vi "Extract Segment.vi"(6 "Containing Type":T2, 8 "error in (no error)":errorcluster, 9 "In Type":bool, 10 "String":string, 11 "ProtoParser in":refnum<class "ProtoParser.lvclass">) -> (0 "error out":errorcluster, 1 "Segment":T1, 2 "Remaining":string, 3 "ProtoParser out":refnum<class "ProtoParser.lvclass">)   [LabVIEW 2020, in "LV-Protoc.lvlib" / "ProtoParser.lvclass"]
uses:
  ProtoParser.lvclass
  Segment Type.ctl
  Raw Segment.ctl
  ProtoParser.lvclass/ProtoParser.ctl
  LV-Protoc.lvlib
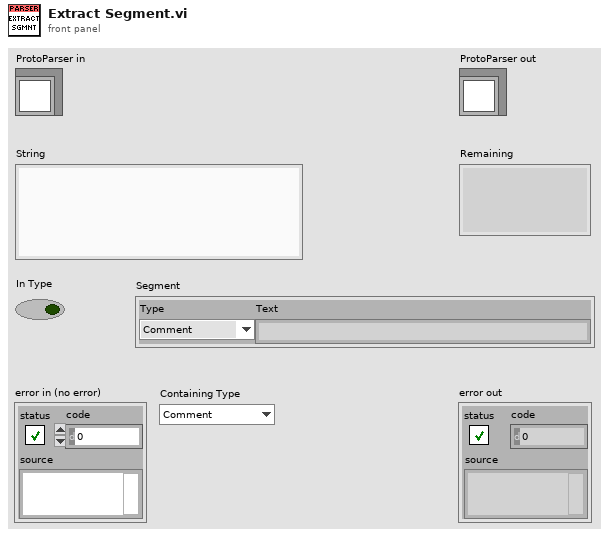
[diagram p1: front panel]
types:
  T1 = typedef "LV-Protoc.lvlib/Raw Segment.ctl" = cluster{"Type":T2, "Text":string}
  T2 = typedef "LV-Protoc.lvlib/Segment Type.ctl" = enum16{"Comment", "Message Open", "Enum Open", "Message Close", "Enum Close", "Field", "Syntax", "Import", "Enum Value", "Package", "Reserved"}
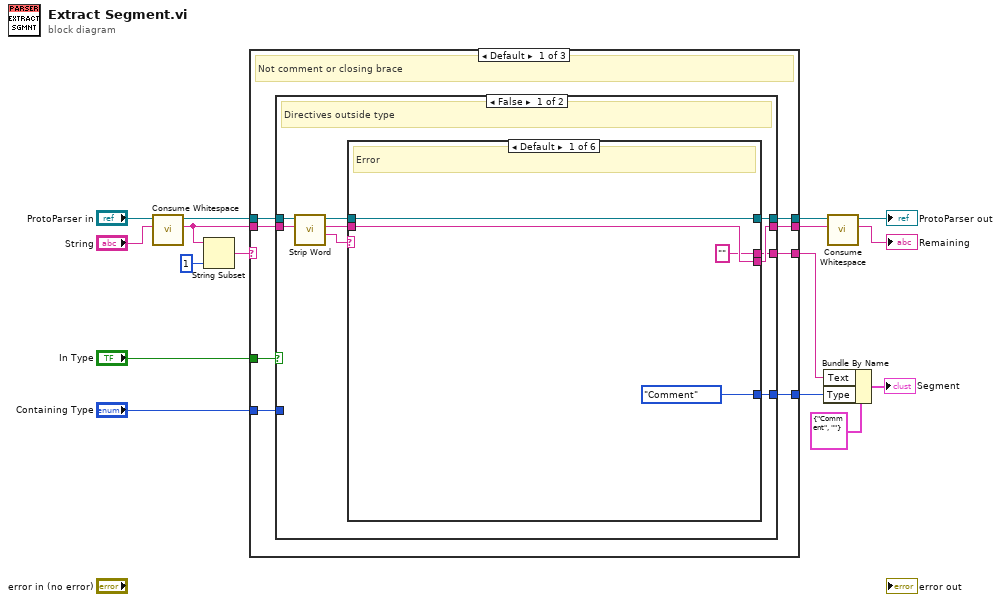
[diagram p0: block diagram]
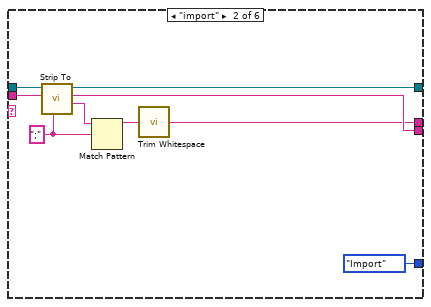
[diagram p2: hidden frame]
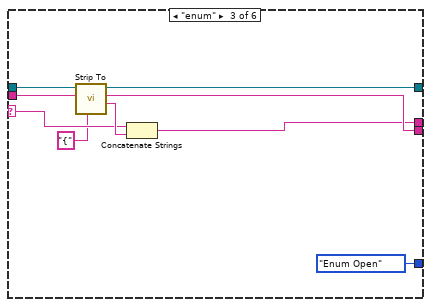
[diagram p3: hidden frame]
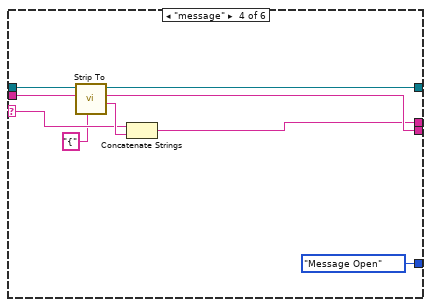
[diagram p4: hidden frame]
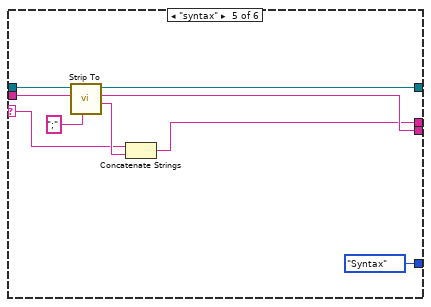
[diagram p5: hidden frame]
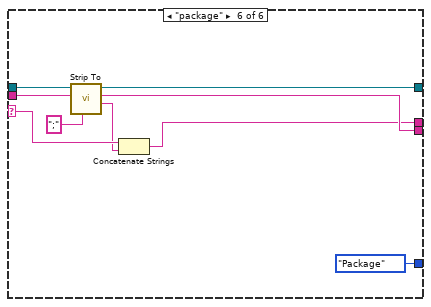
[diagram p6: hidden frame]
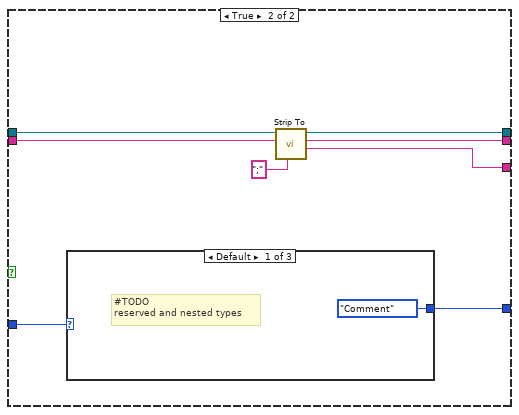
[diagram p7: hidden frame]
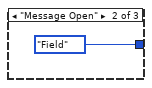
[diagram p8: hidden frame]
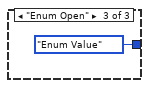
[diagram p9: hidden frame]
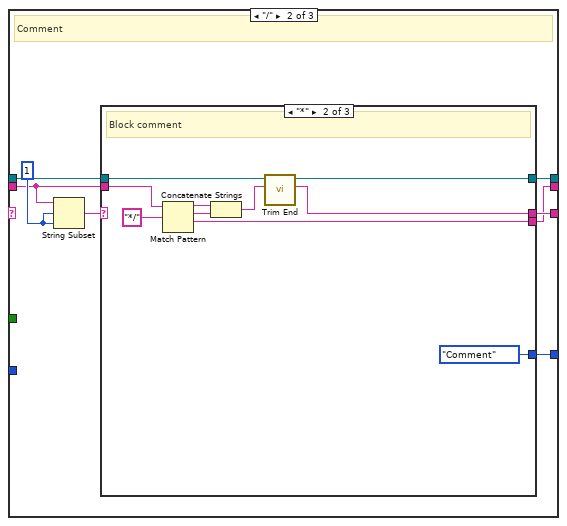
[diagram p10: hidden frame]
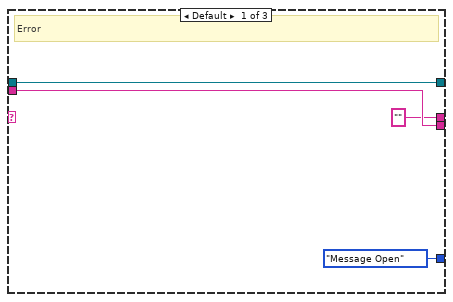
[diagram p11: hidden frame]
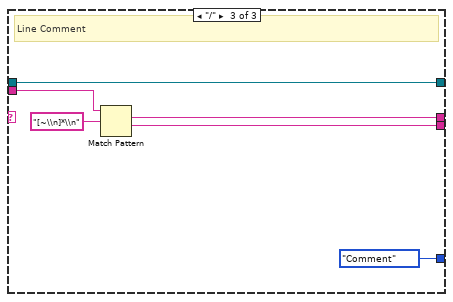
[diagram p12: hidden frame]
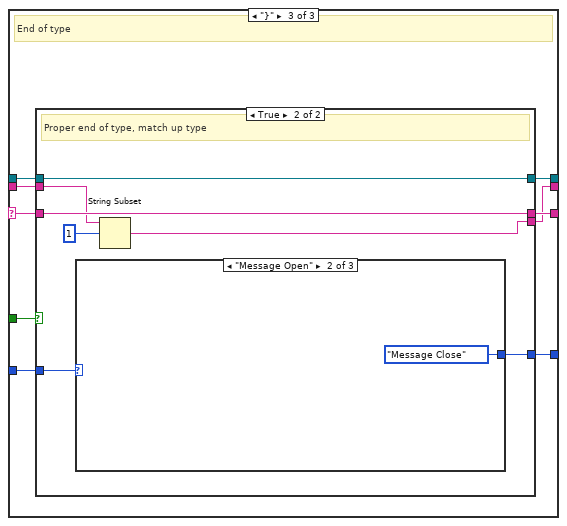
[diagram p13: hidden frame]
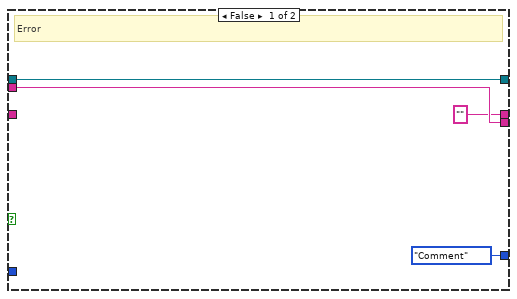
[diagram p14: hidden frame]
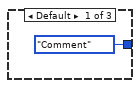
[diagram p15: hidden frame]
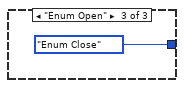
[diagram p16: hidden frame]
diagram:
  n1 = call "Consume Whitespace.vi"("String"="String", "ProtoParser in"="ProtoParser in") -> ("Remaining"=w11:string, "ProtoParser out"=w10:refnum<class "ProtoParser.lvclass">)  [unwired: 7 in, 1 out]
  n2 = String Subset(string=w11, length (rest)=1 ("length (rest)")) -> (substring=w13:string)  [unwired: 1 in]
  n3 = case shown="Default" w13 {
    selector: w13 -> [_ _ w125]
    tunnel: "In Type" -> [w24 _ w128]
    tunnel: w11 -> [w22 w99 w129]
    tunnel: [w18 w98 w124] -> w5
    tunnel: [w17 w97 w126] -> w6
    tunnel: [w19 w96 w122] -> w2
    tunnel: w10 -> [w23 w95 w130]
    tunnel: [w20 w94 w123] -> w4
    tunnel: "Containing Type" -> [w21 _ w127]
    frame Default {
      # "Not comment or closing brace"
      n4 = case shown="False" w24 {
        tunnel: w23 -> [w33 w86]
        tunnel: w22 -> [w32 w85]
        tunnel: w21 -> [_ w84]
        tunnel: [w28 w90] -> w20
        tunnel: [w27 w89] -> w19
        tunnel: [w26 w87] -> w18
        tunnel: [w25 w83] -> w17
        frame False {
          # "Directives outside type"
          n5 = call "Strip Word.vi"("String"=w32, "ProtoParser in"=w33) -> ("Word"=w29:string, "Remaining"=w30:string, "ProtoParser out"=w31:refnum<class "ProtoParser.lvclass">)  [unwired: 6 in, 1 out]
          n6 = case shown="Default" w29 {
            selector: w29 -> [_ _ w50 w59 w66 w76]
            tunnel: w31 -> [w37 w46 w55 w64 w73 w82]
            tunnel: w30 -> [w36 w45 w53 w62 w72 w81]
            tunnel: [w37 w43 w54 w63 w70 w79] -> w28
            tunnel: [w36 w44 w52 w61 w71 w80] -> w27
            tunnel: ["" w39 w49 w58 w65 w74] -> w26
            tunnel: [Segment_Type."Comment" ("Type") Segment_Type."Import" ("Type") Segment_Type."Enum Open" ("Type") Segment_Type."Message Open" ("Type") Segment_Type."Syntax" ("Type") Segment_Type."Package" ("Type")] -> w25
            frame Default {
              # "Error"
            }
            frame "import" {
              w41 = ";" ("End")
              n7 = call "Strip To.vi"("End"=w41, "String"=w45, "ProtoParser in"=w46) -> ("Portion"=w42:string, "Remaining"=w44:string, "ProtoParser out"=w43:refnum<class "ProtoParser.lvclass">)  [unwired: 5 in, 1 out]
              n8 = Match Pattern(string=w42, regular expression=w41) -> (before substring=w40:string)  [unwired: 1 in, 3 out]
              n9 = call <vilib>:"Trim Whitespace.vi"("string"=w40) -> ("trimmed string"=w39:string)  [unwired: 1 in]
            }
            frame "enum" {
              n10 = call "Strip To.vi"("End"="{", "String"=w53, "ProtoParser in"=w55) -> ("Portion"=w51:string, "Remaining"=w52:string, "ProtoParser out"=w54:refnum<class "ProtoParser.lvclass">)  [unwired: 5 in, 1 out]
              n11 = Concatenate Strings(w50, w51) -> (w49:string)
            }
            frame "message" {
              n12 = call "Strip To.vi"("End"="{", "String"=w62, "ProtoParser in"=w64) -> ("Portion"=w60:string, "Remaining"=w61:string, "ProtoParser out"=w63:refnum<class "ProtoParser.lvclass">)  [unwired: 5 in, 1 out]
              n13 = Concatenate Strings(w59, w60) -> (w58:string)
            }
            frame "syntax" {
              n14 = call "Strip To.vi"("End"=";", "String"=w72, "ProtoParser in"=w73) -> ("Portion"=w67:string, "Remaining"=w71:string, "ProtoParser out"=w70:refnum<class "ProtoParser.lvclass">)  [unwired: 5 in, 1 out]
              n15 = Concatenate Strings(w66, w67) -> (w65:string)
            }
            frame "package" {
              n16 = call "Strip To.vi"("End"=";", "String"=w81, "ProtoParser in"=w82) -> ("Portion"=w75:string, "Remaining"=w80:string, "ProtoParser out"=w79:refnum<class "ProtoParser.lvclass">)  [unwired: 5 in, 1 out]
              n17 = Concatenate Strings(w76, w75) -> (w74:string)
            }
          }
        }
        frame True {
          n18 = case shown="Default" w84 {
            tunnel: [Segment_Type."Comment" ("Type") Segment_Type."Field" ("Type") Segment_Type."Enum Value" ("Type")] -> w83
            frame Default {
              # "#TODO\nreserved and nested types"
            }
            frame "Message Open" {
            }
            frame "Enum Open" {
            }
          }
          n19 = call "Strip To.vi"("End"=";", "String"=w85, "ProtoParser in"=w86) -> ("Portion"=w87:string, "Remaining"=w89:string, "ProtoParser out"=w90:refnum<class "ProtoParser.lvclass">)  [unwired: 5 in, 1 out]
        }
      }
    }
    frame "/" {
      w101 = 1 ("offset (0)")
      # "Comment"
      n20 = String Subset(string=w99, offset (0)=w101, length (rest)=w101) -> (substring=w100:string)
      n21 = case shown="\"*\"" w100 {
        tunnel: w99 -> [w103 w114 w121]
        tunnel: ["" ("Remaining") w106 w119] -> w98
        tunnel: [Segment_Type."Message Open" ("Type") Segment_Type."Comment" ("Type") Segment_Type."Comment" ("Type")] -> w97
        tunnel: [w103 w112 w117] -> w96
        tunnel: w95 -> [w105 w115 w116]
        tunnel: [w105 w108 w116] -> w94
        frame Default {
          # "Error"
        }
        frame "*" {
          # "Block comment"
          n22 = Match Pattern(string=w114, regular expression="*/") -> (before substring=w111:string, match substring=w110:string, after substring=w112:string)  [unwired: 1 in, 1 out]
          n23 = Concatenate Strings(w111, w110) -> (w107:string)
          n24 = call "Trim End.vi"("String"=w107, "ProtoParser in"=w115) -> ("Trimmed"=w106:string, "ProtoParser out"=w108:refnum<class "ProtoParser.lvclass">)  [unwired: 7 in, 1 out]
        }
        frame "/" {
          # "Line Comment"
          n25 = Match Pattern(string=w121, regular expression="[~\\n]*\\n") -> (match substring=w119:string, after substring=w117:string)  [unwired: 1 in, 2 out]
        }
      }
    }
    frame "}" {
      # "End of type"
      n26 = case shown="True" w128 {
        tunnel: w130 -> [w134 w138]
        tunnel: w129 -> [w133 w137]
        tunnel: w127 -> [_ w141]
        tunnel: [Segment_Type."Comment" ("Type") w140] -> w126
        tunnel: w125 -> [_ w139]
        tunnel: ["" w139] -> w124
        tunnel: [w134 w138] -> w123
        tunnel: [w133 w135] -> w122
        frame False {
          # "Error"
        }
        frame True {
          # "Proper end of type, match up type"
          n27 = case shown="\"Message Open\"" w141 {
            tunnel: [Segment_Type."Comment" ("Type") Segment_Type."Message Close" ("Type") Segment_Type."Enum Close" ("Type")] -> w140
            frame Default {
            }
            frame "Message Open" {
            }
            frame "Enum Open" {
            }
          }
          n28 = String Subset(string=w137, offset (0)=1) -> (substring=w135:string)  [unwired: 1 in]
        }
      }
    }
  }
  n29 = Bundle By Name(cluster=T1 {"Type"=enum."Comment", "Text"=""} ("Segment"), "Text"=w5, "Type"=w6) -> (→"Segment":T1)
  n30 = call "Consume Whitespace.vi"("String"=w2, "ProtoParser in"=w4) -> ("Remaining"=→"Remaining":string, "ProtoParser out"=→"ProtoParser out":refnum<class "ProtoParser.lvclass">)  [unwired: 7 in, 1 out]
